vi "Get Bitfile Path.vi"(8 "error in (no error)":errorcluster, 10 "SI Count":i32, 11 "Module Name":string) -> (0 "error out":errorcluster, 3 "Bitfile Path":path)   [LabVIEW 2025, in "I2C Bus Monitor UI.lvlib"]
uses:
  I2C Bus Monitor UI.lvlib
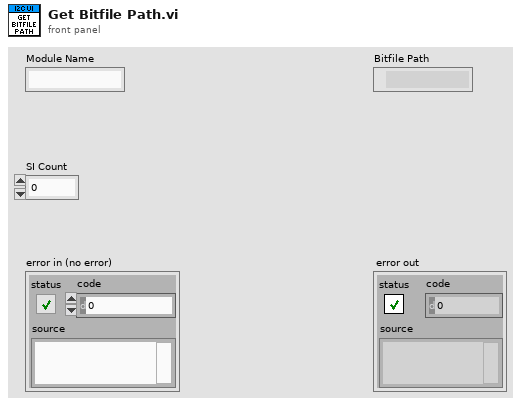
[diagram p1: front panel]
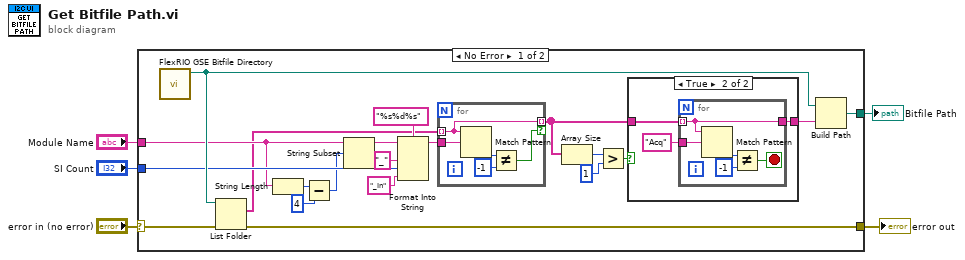
[diagram p0: block diagram]
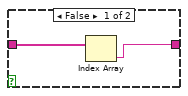
[diagram p2: hidden frame]
diagram:
  n1 = case shown="No Error" "error in (no error)" {
    selector: "error in (no error)" -> [w25 w41]
    tunnel: "SI Count" -> [w16 _]
    tunnel: "Module Name" -> [w9 _]
    tunnel: [w7 _] -> w2
    tunnel: [w6 w41] -> w1
    frame No Error {
      n2 = call "FlexRIO GSE Bitfile Directory.vi"() -> ("Flexrio GSE Template Bitfiles Folder Path"=w23:path)  [unwired: 11 in]
      n3 = List Folder(path=w23, error in=w25) -> (filenames=w8:string[], error out=w6:errorcluster)  [unwired: 2 in, 2 out]
      n4 = String Length(string=w9) -> (length=w10:i32)
      n5 = Subtract(x=w10, y=4) -> (x-y=w11:i32)
      n6 = String Subset(string=w9, offset (0)=w11) -> (substring=w14:string)  [unwired: 1 in]
      n7 = Format Into String(format string="%s%d%s", initial string=w14, "_" ("substring"), w16, "_In" ("substring")) -> (resulting string=w15:string)  [unwired: 1 in, 1 out]
      n8 = for {
        tunnel: w8 -> [w37] mode=indexing
        tunnel: w15 -> [w40]
        tunnel: [w37] -> w22 mode=indexing if=w36
        n9 = Match Pattern(string=w37, regular expression=w40) -> (offset past match=w38:i32)  [unwired: 1 in, 3 out]
        n10 = Not Equal?(x=w38, y=-1) -> (x != y?=w36:bool)
      }
      n11 = Array Size(array=w22) -> (size(s)=w19:i32)
      n12 = Greater?(x=w19, y=1) -> (0:w21:bool)
      n13 = case shown="True" w21 {
        tunnel: w22 -> [w27 w30]
        tunnel: [w26 w28] -> w24
        frame False {
          n14 = Index Array(array=w27) -> (element=w26:string)  [unwired: 1 in]
        }
        frame True {
          n15 = for {
            tunnel: w30 -> [w32] mode=indexing
            tunnel: "Acq" -> [w35]
            tunnel: [w32] -> w28
            stop <- w31 stop-if-true
            n16 = Match Pattern(string=w32, regular expression=w35) -> (offset past match=w33:i32)  [unwired: 1 in, 3 out]
            n17 = Not Equal?(x=w33, y=-1) -> (x != y?=w31:bool)
          }
        }
      }
      n18 = Build Path(base path=w23, name or relative path=w24) -> (appended path=w7:path)
    }
    frame Error {
    }
  }
  "error out" <- w1
  "Bitfile Path" <- w2
